vi "libssh2_agent_sign.vi"(8 "error in (no error)":errorcluster, 9 "data":u8[](array[numeric]), 10 "identity":T1, 11 "agent":T2) -> (0 "error out":errorcluster, 2 "signature":u8[](array[numeric]))   [LabVIEW 2017, in "libssh2.lvlib"]
doc: "Sign a buffer with a public key from an SSH agent."
uses:
  libssh2.lvlib
  Agent Refnum.ctl
  Agent Public Key Refnum.ctl
  Acquire Session.vi
  Release Session.vi
  Not An Agent.vi
  <vilib>/Utility/error.llb/Error Cluster From Error Code.vi
  Not An Agent Public Key.vi
  Global Settings.vi
  Read Agent Refnum.vi
  Read Session Refnum.vi
  <vilib>/Utility/semaphor.llb/Acquire Semaphore.vi
  <vilib>/Utility/semaphor.llb/Release Semaphore.vi
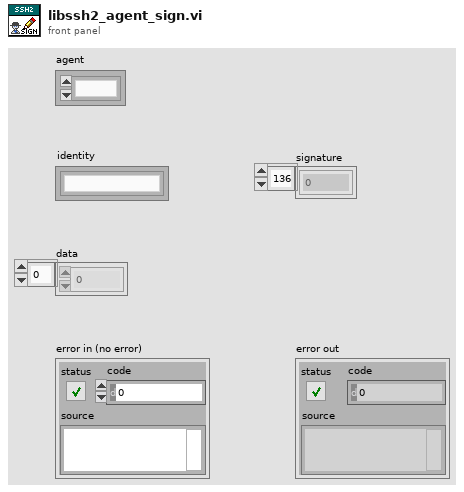
[diagram p1: front panel]
types:
  T1 = typedef "libssh2.lvlib/Agent Public Key Refnum.ctl" = refnum<k1>
  T2 = typedef "libssh2.lvlib/Agent Refnum.ctl" = refnum<k1>
  T3 = typedef "libssh2.lvlib/libssh2_agent_publickey.ctl" = cluster{"magic":u32, "node":u64, "blob":u8[], "blob_len":u64, "comment":string}
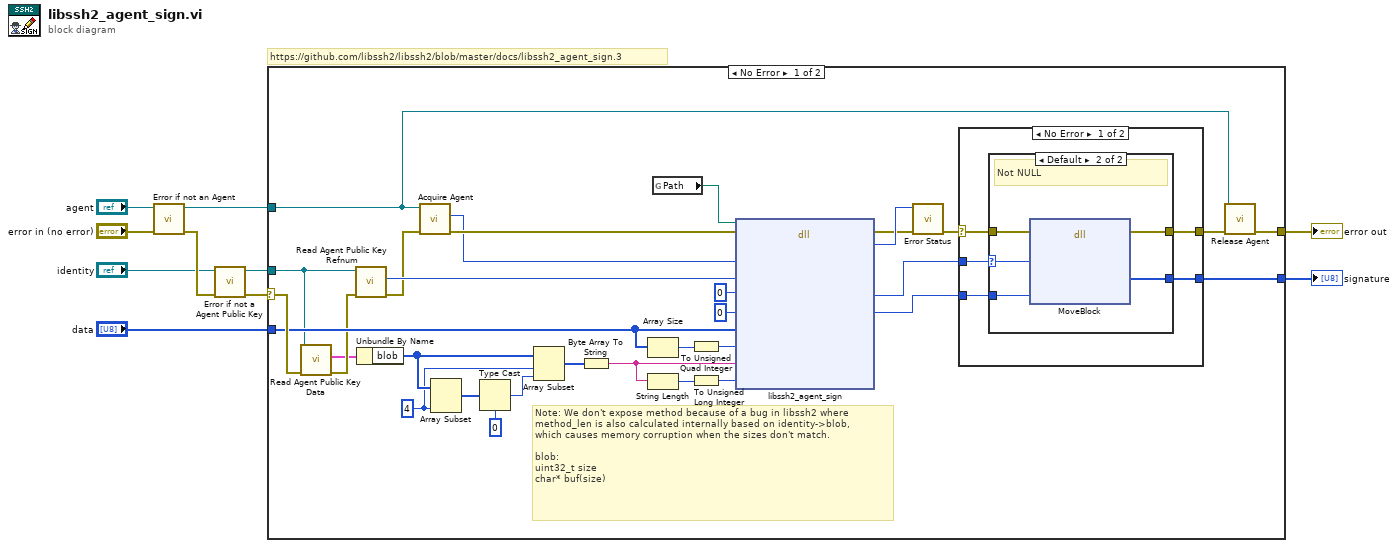
[diagram p0: block diagram]
diagram:
  # "https://github.com/libssh2/libssh2/blob/master/docs/libssh2_agent_sign.3"
  n1 = call "Error if not an Agent.vi"("error in (no error)"="error in (no error)", "agent"="agent") -> ("error out"=w6:errorcluster, "agent out"=w7:T2)  [unwired: 8 in]
  n2 = call "Error if not a Agent Public Key.vi"("error in (no error)"=w6, "agent public key"="identity") -> ("error out"=w5:errorcluster, "agent public key out"=w3:T1)  [unwired: 8 in]
  n3 = case shown="No Error" w5 {
    selector: w5 -> [w37 w54]
    tunnel: [w12 w54] -> w10
    tunnel: w7 -> [w11 _]
    tunnel: w3 -> [w21 _]
    tunnel: "data" -> [w34 _]
    tunnel: [w24 _] -> w1
    frame No Error {
      w15 = 4 ("length")
      # "Note: We don't expose method because of a bug in libssh2 where method_len is also calculated internally based on identity->blob,\nwhich causes memory corruption when the sizes don't match.\n\nblob:\nuint32_t size\nchar* buf(size)"
      n4 = call "Read Agent Public Key Data.vi"("error in (no error)"=w37, "agent public key"=w21) -> ("error out"=w22:errorcluster, "value"=w20:T3)  [unwired: 8 in]
      n5 = call "Read Agent Public Key Refnum.vi"("error in (no error)"=w22, "agent public key"=w21) -> ("error out"=w36:errorcluster, "libssh2_agent_publickey*"=w38:u64)  [unwired: 7 in, 1 out]
      n6 = Unbundle By Name(w20) -> ("blob"=w17:u8[])
      n7 = call "Acquire Agent.vi"("error in (no error)"=w36, "agent"=w11) -> ("error out"=w40:errorcluster, "LIBSSH2_AGENT*"=w39:u64)  [unwired: 8 in]
      n8 = Array Subset(array=w17, length=w15) -> (w19:u8[])  [unwired: 1 in]
      n9 = Type Cast(type=u32 0, x=w19) -> (*(type *) &x=w16:u32)
      n10 = Array Subset(array=w17, index=w15, length=w16) -> (w14:u8[])
      n11 = Byte Array To String(unsigned byte array=w14) -> (string=w13:string)
      n12 = Array Size(array=w34) -> (size(s)=w33:i32)
      n13 = String Length(string=w13) -> (length=w31:i32)
      n14 = global read "Global Settings.vi" "Path"() -> (w41:path)
      n15 = To Unsigned Quad Integer(1:w33) -> (0:w32:u64)
      n16 = To Unsigned Long Integer(number=w31) -> (unsigned 32bit integer=w30:u32)
      n17 = dll-call lib="?" fn="libssh2_agent_sign"(path in=w41, error in=w40, "agent"=w39, "identity"=w38, "sig"=u64 0, "s_len"=u64 0, "data"=w34, "d_len"=w32, "method"=w13, "method_len"=w30) -> (error out=w29:errorcluster, "return value"=w42:i32, "sig"=w27:u64, "s_len"=w26:u64)  [unwired: 7 in, 1 out]
      n18 = call "Error Status.vi"("error in (no error)"=w29, "return value"=w42) -> ("error out"=w23:errorcluster)  [unwired: 8 in, 1 out]
      n19 = case shown="No Error" w23 {
        selector: w23 -> [w43 w53]
        tunnel: w27 -> [w47 _]
        tunnel: w26 -> [w46 _]
        tunnel: [w45 w53] -> w25
        tunnel: [w44 _] -> w24
        frame No Error {
          n20 = case shown="Default" w47 {
            selector: w47 -> [_ w49]
            tunnel: w46 -> [_ w52]
            tunnel: [_ w51] -> w44
            tunnel: [_ w50] -> w45
            tunnel: w43 -> [_ w48]
            frame 0 {
              # "NULL"
            }
            frame Default {
              # "Not NULL"
              n21 = dll-call lib="LabVIEW" fn="MoveBlock"(error in=w48, "ps"=w49, "size"=w52) -> (error out=w50:errorcluster, "pd"=w51:u8[])  [unwired: 6 in, 1 out]
            }
          }
        }
        frame Error {
        }
      }
      n22 = call "Release Agent.vi"("error in (no error)"=w25, "agent"=w11) -> ("error out"=w12:errorcluster)  [unwired: 9 in]
    }
    frame Error {
    }
  }
  "error out" <- w10
  "signature" <- w1
